vi "test1-ModuleCreatedDestroyed_Queue.vi"(8 "error in (no error)":errorcluster, 11 "TestCase in":refnum<class "testcase-CSMGlobalLog.lvclass">) -> (0 "error out":errorcluster, 3 "TestCase out":refnum<class "testcase-CSMGlobalLog.lvclass">)   [LabVIEW 2017, in "testcase-CSMGlobalLog.lvclass"]
uses:
  testcase-CSMGlobalLog.lvclass
  testcase-CSMGlobalLog.lvclass/testcase-CSMGlobalLog.ctl
  64b6e408-f0cd-4aee-a387-1a6bb95babb2.vi
  <vilib>/addons/_JKI Toolkits/VI Tester/TestCase.llb/TestCase.lvclass
  src/user.lib/_NEVSTOP/Communicable State Machine(CSM)/Utility/Periodic String Filter Setting.ctl
  src/user.lib/_NEVSTOP/Communicable State Machine(CSM)/Communicable State Machine.lvlib
  C:/Program Files (x86)/National Instruments/LabVIEW 2017/vi.lib/addons/_JKI Toolkits/VI Tester/TestCase.llb/TestCase.lvclass
panel:
  out "String Cache Each Loop":string
  out "String cache total":string
  out "LoopCount":i32
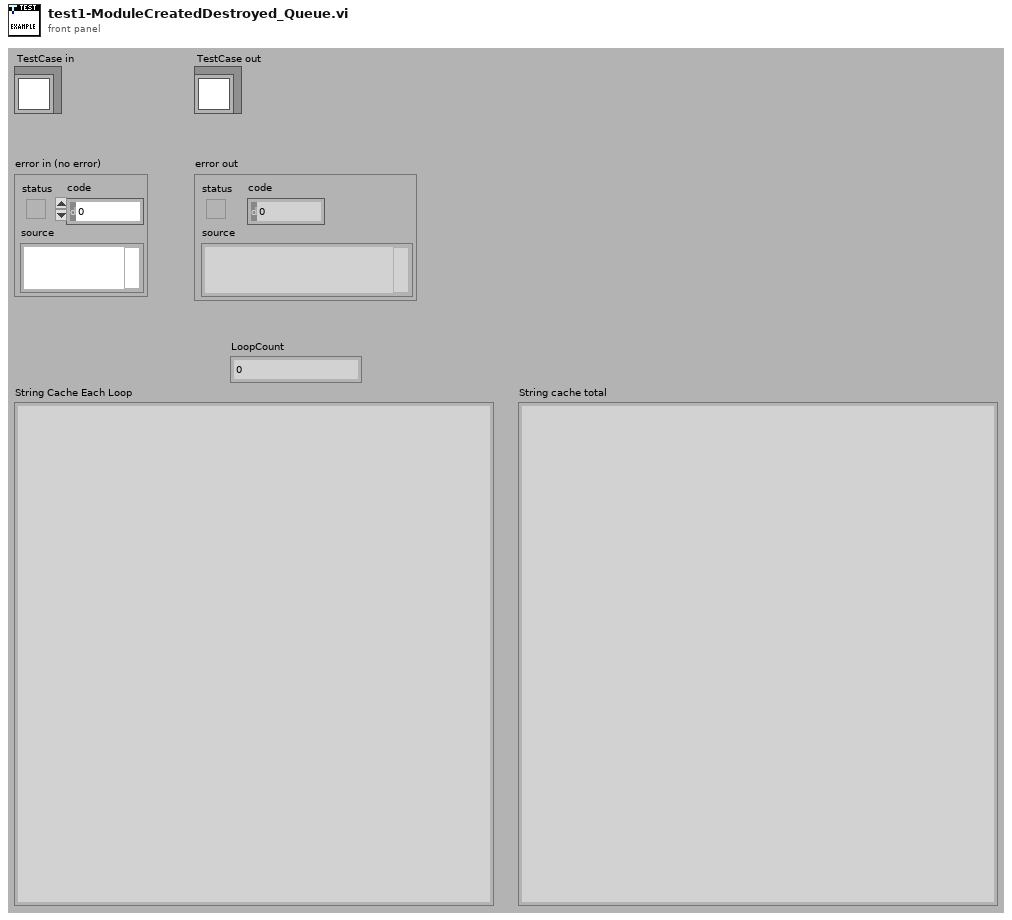
[diagram p1: front panel]
types:
  T1 = typedef "Communicable State Machine.lvlib/Periodic String Filter Setting.ctl" = cluster{"threashold(#/s)":dbl, "Check Peroid(s)":dbl}
  T2 = typedef "Communicable State Machine.lvlib/_CSM_GlobalLog_MSG.ctl" = cluster{"Name (\"\" to Use UUID)":string, "Current State":string, "Arguments":string, "Source Message":T3, "Source Module":string, "Complete(T)/Start(F)":bool, "LogType":T4, "Time Stamp":timestamp}
  T3 = typedef "Communicable State Machine.lvlib/_CSM_Response Source Message.ctl" = cluster{"‘State":string, "’Arguments":string, "’Error":errorcluster}
  T4 = typedef "Communicable State Machine.lvlib/_CSM_GlobalLog_MSG_TYPE.ctl" = enum16{"User Log", "State Change", "Status", "Interrupt", "Register", "Unregister", "Error Log", "Module Created", "Module Destroyed", "Async Message", "No-Rep Async Message", "Sync Message"}
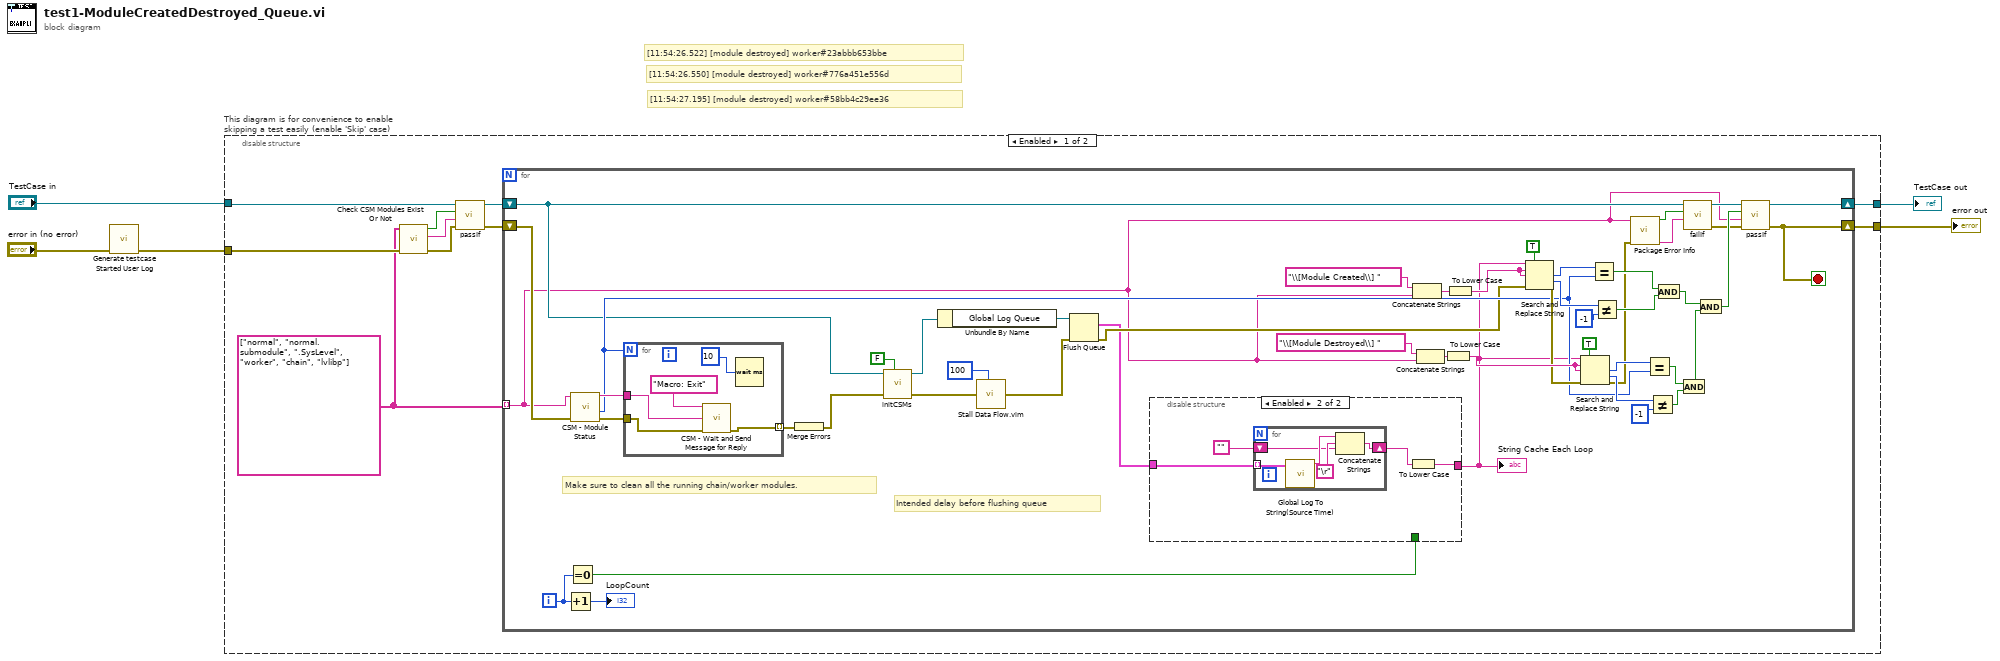
[diagram p0: block diagram]
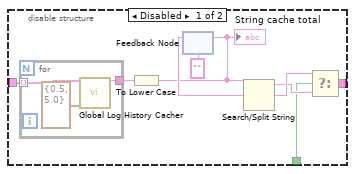
[diagram p2: hidden frame]
diagram:
  # "[11:54:26.522] [module destroyed] worker#23abbb653bbe"
  # "[11:54:27.195] [module destroyed] worker#58bb4c29ee36"
  # "[11:54:26.550] [module destroyed] worker#776a451e556d"
  n1 = call "Generate testcase Started User Log.vi"("Error In"="error in (no error)") -> ("error out"=w1:errorcluster)  [unwired: 10 in]
  n2 = disable-structure "This diagram is for convenience to enable skipping a test easily (enable 'Skip' case)" shown="Enabled" {
    disable-tunnel: "TestCase in" -> [w10 w94]
    disable-tunnel: [w14 w92] -> w2
    disable-tunnel: [w15 w93] -> w4
    disable-tunnel: w1 -> [w8 w91]
    frame Enabled {
      w6 = string[] ["normal", "normal.submodule", ".SysLevel", "worker", "chain", "lvlibp"]
      n3 = call "Check CSM Modules Exist Or Not.vi"("error in"=w8, "CSM names in"=w6) -> ("error out"=w11:errorcluster, "Debug string"=w12:string, "All Modules Exist?"=w13:bool)  [unwired: 7 in]
      n4 = call-dynamic "passIf.vi"("error in (no error)"=w11, "message (\"\")"=w12, "pass"=w13, "TestCase in"=w10) -> ("error out"=w7:errorcluster, "TestCase out"=w9:refnum<class "testcase-CSMGlobalLog.lvclass">)  [unwired: 6 in]
      n5 = for {
        tunnel: w6 -> [w16] mode=indexing
        shift-right: [w32] -> w15
        shift-left: w7 -> [w24]
        shift-right: [w64] -> w14
        shift-left: w9 -> [w20]
        i -> [w26]
        stop <- w32 stop-if-true
        # "Intended delay before flushing queue"
        # "Make sure to clean all the running chain/worker modules."
        n6 = Increment(x=w26) -> (x+1=→"LoopCount":i32)
        n7 = Equal To 0?(x=w26) -> (x = 0?=w25:bool)
        n8 = call "CSM - Module Status.vi"("Error In"=w24, "CSM Name"=w16) -> ("error out"=w23:errorcluster, "#Nodes"=w39:i32, "CSM Name (Dup)"=w56:string)  [unwired: 5 in, 2 out]
        n9 = for {
          N: w39 -> [_]
          tunnel: [w89] -> w55 mode=indexing
          tunnel: w56 -> [w88]
          tunnel: w23 -> [w87]
          n10 = call "CSM - Wait and Send Message for Reply.vi"("State"="Macro: Exit", "Target Module"=w88, "Error In (No Error)"=w87) -> ("error out"=w89:errorcluster)  [unwired: 9 in, 3 out]
          n11 = Wait (ms)(milliseconds to wait=u32 10) -> ()  [unwired: 1 out]
        }
        n12 = Merge Errors(w55) -> (w34:errorcluster)
        n13 = call "initCSMs.vi"("Enable building lvlibp?"=FALSE, "error in (no error)"=w34, "TestCase in"=w20) -> ("error out"=w31:errorcluster, "TestCase out"=w33:refnum<class "testcase-CSMGlobalLog.lvclass">)  [unwired: 7 in]
        n14 = Unbundle By Name(w33) -> ("Global Log Queue"=w63:refnum<queue>)
        n15 = call "Stall Data Flow.vim"("value in"=w31, "milliseconds to wait"=u32 100) -> ("value out"=w30:errorcluster)  [unwired: 1 out]
        n16 = Flush Queue(queue=w63, error in (no error)=w30) -> (remaining elements=w28:T2[], error out=w35:errorcluster)  [unwired: 1 out]
        n17 = disable-structure shown="Enabled" {
          disable-tunnel: [w67 w77] -> w27
          disable-tunnel: w25 -> [w66 _]
          disable-tunnel: w28 -> [w65 w79]
          frame Disabled {
            n18 = for {
              tunnel: w65 -> [w76] mode=indexing
              tunnel: [w75] -> w73
              n19 = call "Global Log History Cacher.vi"("Global Log Data"=w76, "Settings"=T1 {"threashold(#/s)"=0.5, "Check Peroid(s)"=5.0}) -> ("String Cache"=w75:string)  [unwired: 13 in]
            }
            n20 = To Lower Case(string=w73) -> (all lower case string=w68:string)
            "String cache total" <- w68
            n21 = feedback #1("") -> (w72:string)
            n22 = feedback-in #1(w68) -> ()
            n23 = Search/Split String(string=w68, search string/char (-)=w72) -> (substring before match=w69:string, match + rest of string=w70:string)  [unwired: 1 in, 1 out]
            n24 = Select(t=w70, s=w66, f=w69) -> (s? t:f=w67:string)
          }
          frame Enabled {
            n25 = for {
              tunnel: w79 -> [w85] mode=indexing
              shift-right: [w81] -> w78
              shift-left: "" -> [w82]
              n26 = call "Global Log To String(Source Time).vi"("Log"=w85) -> ("Log String"=w84:string)  [unwired: 9 in]
              n27 = Concatenate Strings(w84, "\r", w82) -> (w81:string)
            }
            n28 = To Lower Case(string=w78) -> (all lower case string=w77:string)
          }
        }
        "String Cache Each Loop" <- w27
        n29 = Concatenate Strings("\\[Module Created\\] " ("regular expression"), w16) -> (w57:string)
        n30 = Concatenate Strings("\\[Module Destroyed\\] " ("regular expression"), w16) -> (w59:string)
        n31 = To Lower Case(string=w59) -> (all lower case string=w41:string)
        n32 = To Lower Case(string=w57) -> (all lower case string=w53:string)
        n33 = Search and Replace String(replace all?=TRUE ("replace all? (F)"), input string=w27, search string=w53, replace string=w53, error in=w35) -> (number of replacements=w52:i32, offset past replacement=w51:i32, error out=w40:errorcluster)  [unwired: 3 in, 1 out]
        n34 = Search and Replace String(replace all?=TRUE ("replace all? (F)"), input string=w27, search string=w41, replace string=w41, error in=w40) -> (number of replacements=w43:i32, offset past replacement=w44:i32, error out=w17:errorcluster)  [unwired: 3 in, 1 out]
        n35 = Equal?(x=w52, y=w39) -> (x = y?=w49:bool)
        n36 = Not Equal?(x=w51, y=-1) -> (x != y?=w48:bool)
        n37 = call "Package Error Info.vi"("error in"=w17, "String in"=w16) -> ("packed error info out"=w21:string, "error status"=w22:bool)  [unwired: 8 in]
        n38 = Equal?(x=w43, y=w39) -> (x = y?=w46:bool)
        n39 = Not Equal?(x=w44, y=-1) -> (x != y?=w47:bool)
        n40 = And(x=w49, y=w48) -> (x .and. y?=w38:bool)
        n41 = And(x=w46, y=w47) -> (x .and. y?=w37:bool)
        n42 = call-dynamic "failIf.vi"("message (\"\")"=w21, "fail"=w22, "TestCase in"=w20) -> ("error out"=w18:errorcluster, "TestCase out"=w19:refnum<class "testcase-CSMGlobalLog.lvclass">)  [unwired: 7 in]
        n43 = And(x=w38, y=w37) -> (x .and. y?=w36:bool)
        n44 = call-dynamic "passIf.vi"("error in (no error)"=w18, "message (\"\")"=w16, "pass"=w36, "TestCase in"=w19) -> ("error out"=w32:errorcluster, "TestCase out"=w64:refnum<class "testcase-CSMGlobalLog.lvclass">)  [unwired: 6 in]
      }
    }
    frame Disabled {
      # "skip test result while test is under development"
      n45 = call <vilib>:"skip.vi"("error in (no error)"=w91, "TestCase in"=w94) -> ("error out"=w93:errorcluster, "TestCase out"=w92:refnum<class "testcase-CSMGlobalLog.lvclass">)  [unwired: 8 in]
    }
  }
  "error out" <- w4
  "TestCase out" <- w2
